vi "Check IDN.vi"(8 "error in":errorcluster, 11 "VISA Refnum in":refnum<visa-resource-name>) -> (0 "error out":errorcluster, 2 "IDN OK?":bool, 3 "VISA Refnum out":refnum<visa-resource-name>)   [LabVIEW 2019, in "DAC.lvlib" / "DAC HMP4040.lvclass"]
uses:
  DAC HMP4040.lvclass
  7b33573d-7855-4d2e-99d3-3788cab70eb5.vi
  49045042-62d0-4bb2-8d80-2c7de03f5420.vi
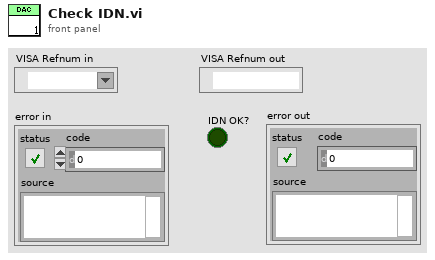
[diagram p1: front panel]
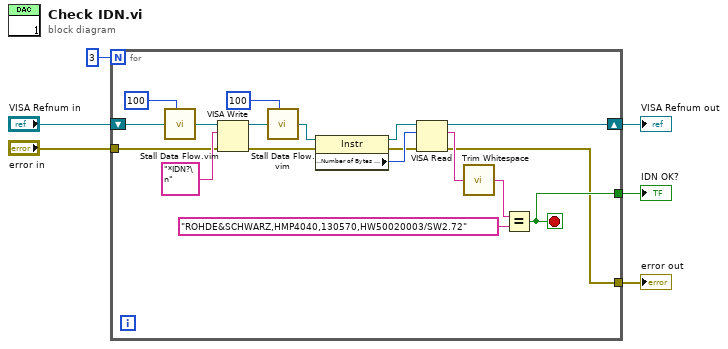
[diagram p0: block diagram]
diagram:
  n1 = for {
    N: 3 -> [_]
    tunnel: "error in" -> [w16]
    shift-right: [w15] -> w6
    shift-left: "VISA Refnum in" -> [w9]
    tunnel: [w10] -> w2
    tunnel: [w7] -> w1
    stop <- w10 stop-if-true
    n2 = call "Stall Data Flow.vim"("value in"=w9, "milliseconds to wait"=u32 100) -> ("value out"=w8:refnum<visa-resource-name>)  [unwired: 1 out]
    n3 = VISA Write(VISA resource name=w8, write buffer="*IDN?\n", error in (no error)=w16) -> (VISA resource name out=w19:refnum<visa-resource-name>, error out=w21:errorcluster)  [unwired: 1 out]
    n4 = call "Stall Data Flow.vim"("value in"=w19, "milliseconds to wait"=u32 100) -> ("value out"=w18:refnum<visa-resource-name>)  [unwired: 1 out]
    n5 = property class="Instr"(reference=w18, error in=w21) -> (reference out=w24:refnum<visa-resource-name>, error out=w22:errorcluster, "Serial Settings:Number of Bytes at Serial Port"=w23:u32)
    n6 = VISA Read(VISA resource name=w24, byte count=w23, error in (no error)=w22) -> (VISA resource name out=w15:refnum<visa-resource-name>, read buffer=w14:string, error out=w7:errorcluster)  [unwired: 1 out]
    n7 = call <vilib>:"Trim Whitespace.vi"("string"=w14) -> ("trimmed string"=w13:string)  [unwired: 1 in]
    n8 = Equal?(x=w13, y="ROHDE&SCHWARZ,HMP4040,130570,HW50020003/SW2.72") -> (x = y?=w10:bool)
  }
  "VISA Refnum out" <- w6
  "IDN OK?" <- w2
  "error out" <- w1
